vi "macro_CreatePathTraj.vi"() -> ()   [LabVIEW 2019, in "PathPlanner24.lvlib"]
uses:
  PathPlanner24.lvlib
  <vilib>/Rock Robotics/WPI/ThirdParty/JAS_Junk/TrajLib/Trajectory_Library.lvlib
  <vilib>/Rock Robotics/WPI/ThirdParty/JAS_Junk/TrajLib/TypeDef/TRANSLATION2D.ctl
  <vilib>/Rock Robotics/WPI/ThirdParty/JAS_Junk/TrajLib/TypeDef/ROTATION2D.ctl
  TypeDef/PathPlannerPathConstraints.ctl
  TypeDef/PathPlannerTrajectoryState.ctl
  TypeDef/PathPlannerTrajectory.ctl
panel:
  out "PathPlannerTrajectory":T1 {"States"."TargetHolonomicRotation"."SIN" format="%13.4f"; "States"."TargetHolonomicRotation"."COS" format="%13.4f"; "States"."TargetHolonomicRotation"."VALUE" format="%13.4f"; "States"."Heading"."SIN" format="%13.4f"; "States"."Heading"."COS" format="%13.4f"; "States"."Heading"."VALUE" format="%13.4f"; "States"."PositionMeters"."Y" format="%14.3f"; "States"."PositionMeters"."X" format="%14.3f"}
  out "Path\nCreation\nError":bool
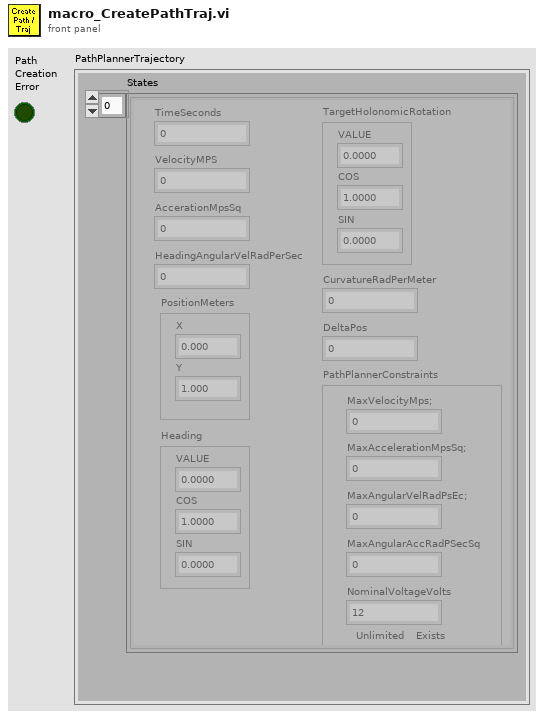
[diagram p1: front panel]
types:
  T1 = typedef "PathPlanner24.lvlib/PathPlannerTrajectory.ctl" = cluster{"States":T2[]}
  T2 = typedef "PathPlanner24.lvlib/PathPlannerTrajectoryState.ctl" = cluster{"TimeSeconds":dbl, "VelocityMPS":dbl, "AccerationMpsSq":dbl, "HeadingAngularVelRadPerSec":dbl, "PositionMeters":T3, "Heading":T4, "TargetHolonomicRotation":T4, "CurvatureRadPerMeter":dbl, "PathPlannerConstraints":T5, "DeltaPos":dbl}
  T3 = typedef "Trajectory_Library.lvlib/TRANSLATION2D.ctl" = cluster{"X":dbl, "Y":dbl}
  T4 = typedef "Trajectory_Library.lvlib/ROTATION2D.ctl" = cluster{"VALUE":dbl, "COS":dbl, "SIN":dbl}
  T5 = typedef "PathPlanner24.lvlib/PathPlannerPathConstraints.ctl" = cluster{"MaxVelocityMps;":dbl, "MaxAccelerationMpsSq;":dbl, "MaxAngularVelRadPsEc;":dbl, "MaxAngularAccRadPSecSq":dbl, "Exists":bool, "Unlimited":bool, "NominalVoltageVolts":dbl}
  T6 = typedef "Trajectory_Library.lvlib/POSE2D.ctl" = cluster{"TRANSLATION":T3, "ROTATION":T4}
  T7 = typedef "Trajectory_Library.lvlib/CHASSIS_SPEEDS.ctl" = cluster{"vX":dbl, "vY":dbl, "vOmega":dbl}
  T8 = typedef "PathPlanner24.lvlib/PathPlannerGoalEndState.ctl" = cluster{"VelocityMPS":dbl, "Rotation":T4}
  T9 = typedef "PathPlanner24.lvlib/PathPlannerWaypoint.ctl" = cluster{"prevControl":T3, "anchor":T3, "nextControl":T3, "PrevExists":bool, "NextExists":bool}
  T10 = typedef "PathPlanner24.lvlib/PathPlannerPath.ctl" = cluster{"Reversed":bool, "RotationTargets":T11[], "ConstraintZones":T12[], "EventMarkers":T13[], "GlobalConstraints":T5, "GoalEndState":T8, "AllPoints":T16[], "Name":string, "Waypoints":T9[], "PointTowardsZones":T17[], "IdealStartingState":T18, "IsChoreoPath":bool, "PreventFlipping":bool}
  T11 = typedef "PathPlanner24.lvlib/PathPlannerRotationTarget.ctl" = cluster{"position":dbl, "rotation":T4, "Exists":bool}
  T12 = typedef "PathPlanner24.lvlib/PathPlannerConstraintsZone.ctl" = cluster{"minPosition":dbl, "maxPosition":dbl, "Constraints":T5, "Present":bool}
  T13 = typedef "PathPlanner24.lvlib/PathPlannerEventMarker.ctl" = cluster{"Position":dbl, "Command":T14, "TriggerName":string, "EndPosition":dbl}
  T14 = typedef "PathPlanner24.lvlib/PathPlannerCommandUtil.ctl" = cluster{"waitTime":dbl, "name":string, "pathName":string, "commands":cluster{"type":T15, "waitTime":dbl, "name":string, "pathName":string}[], "type":T15}
  T15 = typedef "PathPlanner24.lvlib/PathPlanner_CommandUtilType_ENUM.ctl" = enum16{"Unknown", "Wait", "Named", "Path", "Sequential", "Parallel", "Race", "Deadline"}
  T16 = typedef "PathPlanner24.lvlib/PathPlannerPathPoint.ctl" = cluster{"Position":T3, "DistAlongPath":dbl, "MaxV":dbl, "Constraints":T5, "RotationTarget":T11, "WaypointRelativePos":dbl}
  T17 = typedef "PathPlanner24.lvlib/PathPlannerPointTowardsZone.ctl" = cluster{"RotationOffset":T4, "Name":string, "TargetPosition":T3, "MinPosition":dbl, "MaxPosition":dbl}
  T18 = typedef "PathPlanner24.lvlib/PathPlannerIdealStartingState.ctl" = cluster{"VelocityMPS":dbl, "Rotation":T4}
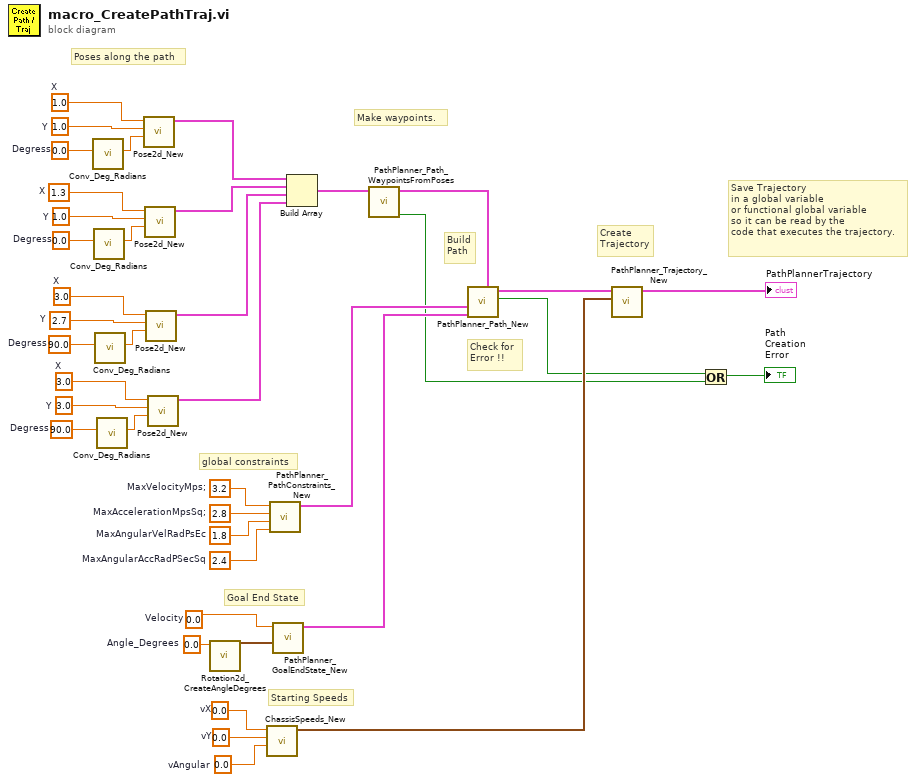
[diagram p0: block diagram]
diagram:
  w7 = 0.0  # vX
  w8 = 0.0  # vY
  w9 = 0.0  # vAngular
  w13 = 0.0  # Angle_Degrees
  w15 = 0.0  # Velocity
  w17 = 3.2  # MaxVelocityMps;
  w18 = 2.8  # MaxAccelerationMpsSq;
  w19 = 1.8  # MaxAngularVelRadPsEc
  w20 = 2.4  # MaxAngularAccRadPSecSq
  w25 = 3.0  # X
  w26 = 3.0  # Y
  w27 = 90.0  # Degress
  w29 = 3.0  # X
  w30 = 2.7  # Y
  w31 = 90.0  # Degress
  w33 = 1.3  # X
  w34 = 1.0  # Y
  w35 = 0.0  # Degress
  w37 = 1.0  # X
  w38 = 1.0  # Y
  w39 = 0.0  # Degress
  # "Save Trajectory\nin a global variable\nor functional global variable\nso it can be read by the \ncode that executes the trajectory."
  # "Create\nTrajectory"
  # "Check for\nError !!"
  # "Starting Speeds"
  # "Goal End State"
  # "global constraints"
  # "Make waypoints."
  # "Build\nPath"
  # "Poses along the path"
  n1 = call <vilib>:"Conv_Deg_Radians.vi"("Degress"=w39) -> ("Radians"=w40:dbl)  [unwired: 10 in]
  n2 = call <vilib>:"Conv_Deg_Radians.vi"("Degress"=w35) -> ("Radians"=w36:dbl)  [unwired: 10 in]
  n3 = call <vilib>:"Conv_Deg_Radians.vi"("Degress"=w31) -> ("Radians"=w32:dbl)  [unwired: 10 in]
  n4 = call <vilib>:"Conv_Deg_Radians.vi"("Degress"=w27) -> ("Radians"=w28:dbl)  [unwired: 10 in]
  n5 = call <vilib>:"Pose2d_New.vi"("Heading"=w40, "Y"=w38, "X"=w37) -> ("out POSe"=w24:T6)  [unwired: 8 in]
  n6 = call <vilib>:"Pose2d_New.vi"("Heading"=w36, "Y"=w34, "X"=w33) -> ("out POSe"=w23:T6)  [unwired: 8 in]
  n7 = call <vilib>:"Pose2d_New.vi"("Heading"=w32, "Y"=w30, "X"=w29) -> ("out POSe"=w22:T6)  [unwired: 8 in]
  n8 = call <vilib>:"Pose2d_New.vi"("Heading"=w28, "Y"=w26, "X"=w25) -> ("out POSe"=w21:T6)  [unwired: 8 in]
  n9 = call <vilib>:"Rotation2d_CreateAngleDegrees.vi"("Angle_Degrees"=w13) -> ("ROTATION"=w14:T4)  [unwired: 10 in]
  n10 = call <vilib>:"ChassisSpeeds_New.vi"("vAngular"=w9, "vY"=w8, "vX"=w7) -> ("CHASSIS"=w6:T7)  [unwired: 8 in]
  n11 = call "PathPlanner_PathConstraints_New.vi"("MaxAngularAccRadPSecSq"=w20, "MaxAngularVelRadPsEc;"=w19, "MaxAccelerationMpsSq;"=w18, "MaxVelocityMps;"=w17) -> ("PathPlannerConstraints"=w16:T5)  [unwired: 7 in]
  n12 = call "PathPlanner_GoalEndState_New.vi"("Rotation"=w14, "VelocityMPS"=w15) -> ("GoalEndState"=w12:T8)  [unwired: 9 in]
  n13 = Build Array(w24, w23, w22, w21) -> (w5:T6[])
  n14 = call "PathPlanner_Path_WaypointsFromPoses.vi"("Poses"=w5) -> ("Error"=w2:bool, "Waypoints"=w4:T9[])  [unwired: 9 in]
  n15 = call "PathPlanner_Path_New.vi"("Waypoints"=w4, "GoalEndState"=w12, "GlobalConstraints"=w16) -> ("Error"=w1:bool, "PathPlannerPath"=w11:T10)  [unwired: 7 in]
  n16 = call "PathPlanner_Trajectory_New.vi"("StartingSpeeds"=w6, "Path"=w11) -> ("PathPlannerTrajectory"=→"PathPlannerTrajectory":T1)  [unwired: 8 in, 1 out]
  n17 = Or(x=w1, y=w2) -> (x .or. y?=→"Path\nCreation\nError":bool)
